vi "Lossy Enqueue Probe I32.vi"(0 "first":i32, 5 "second":i32, 11 "error in":errorcluster) -> (4 "overflow element":i32, 6 "overflow?":bool, 8 "remaining elements":i32[](array[numeric]), 15 "error out":errorcluster)   [LabVIEW 2026]
doc: "Probe: a size-1 queue takes first, then second through Lossy Enqueue Element; the second overflows first out."
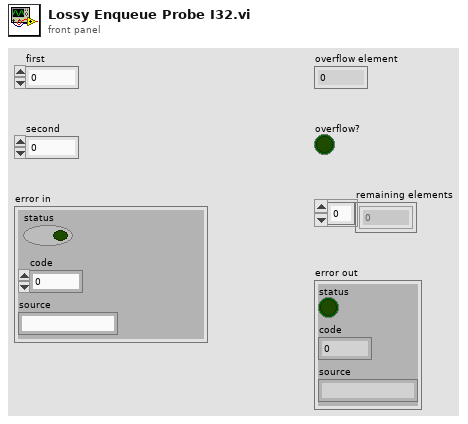
[diagram p1: front panel]
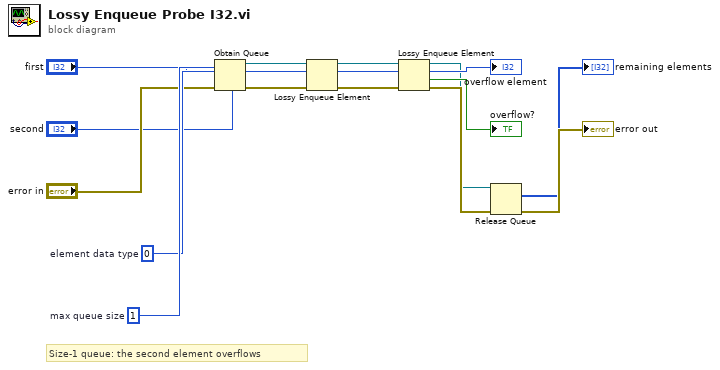
[diagram p0: block diagram]
diagram:
  w5 = 1  # max queue size
  w4 = 0  # element data type
  # "Size-1 queue: the second element overflows"
  n1 = Obtain Queue(max queue size (-1, unlimited)=w5, element data type=w4, error in (no error)="error in") -> (queue out=w6:refnum<queue>, error out=w7:errorcluster)  [unwired: 2 in, 1 out]
  n2 = Lossy Enqueue Element(queue=w6, element="first", error in (no error)=w7) -> (queue out=w8:refnum<queue>, error out=w9:errorcluster)  [unwired: 2 out]
  n3 = Lossy Enqueue Element(queue=w8, element="second", error in (no error)=w9) -> (queue out=w10:refnum<queue>, overflow element=→"overflow element":i32, overflow?=→"overflow?":bool, error out=w13:errorcluster)
  n4 = Release Queue(queue=w10, error in (no error)=w13) -> (remaining elements=→"remaining elements":i32[], error out=→"error out":errorcluster)  [unwired: 1 in, 1 out]
